vi "set Marker Control Mode.vi"(8 "error in (no error)":errorcluster, 9 "Marker Index":i32, 10 "Marker Mode":T1, 11 "FSV-40N in":refnum<class "FSV-40N.lvclass">) -> (0 "error out":errorcluster, 3 "FSV-40N out":refnum<class "FSV-40N.lvclass">)   [LabVIEW 2023, in "Spectrum Analyzer.lvlib" / "FSV-40N.lvclass"]
uses:
  FSV-40N.lvclass
  FSV-40N.lvclass/FSV-40N.ctl
  TYPE DEFINITION/TYPE Marker Control Mode.ctl
  Spectrum Analyzer.lvlib
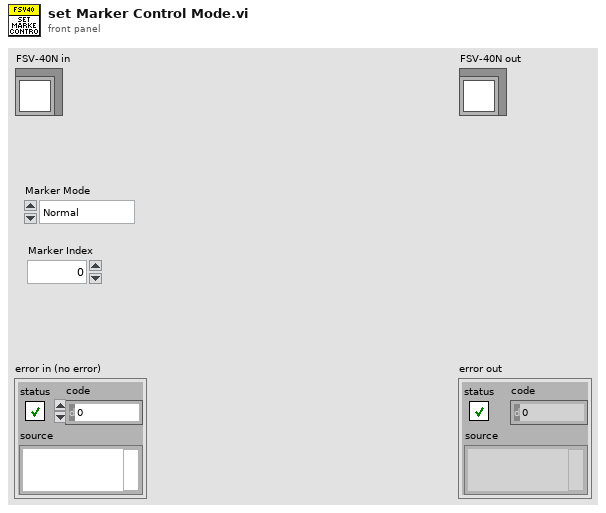
[diagram p1: front panel]
types:
  T1 = typedef "Spectrum Analyzer.lvlib/TYPE Marker Control Mode.ctl" = enum16{"Normal", "Delta", "Off"}
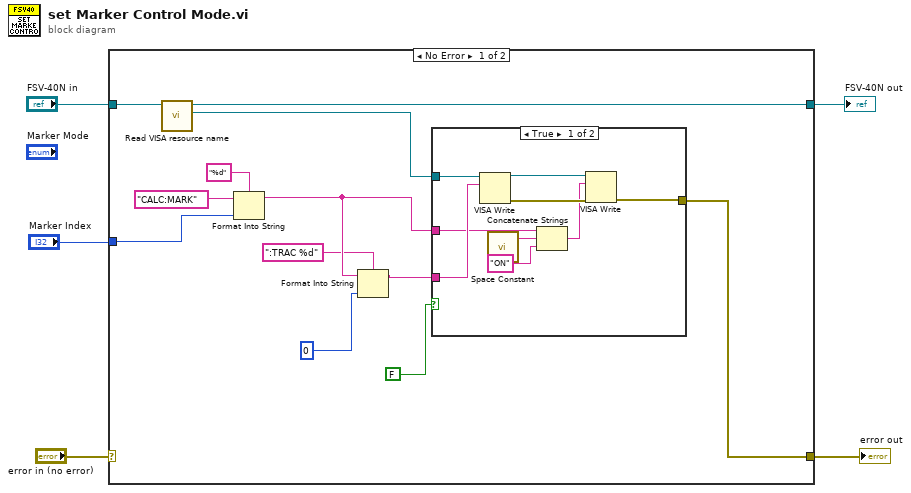
[diagram p0: block diagram]
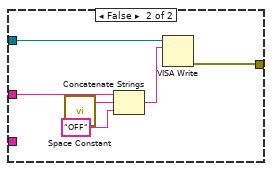
[diagram p2: hidden frame]
diagram:
  n1 = case shown="No Error" "error in (no error)" {
    selector: "error in (no error)" -> [_ w33]
    tunnel: "FSV-40N in" -> [w17 w34]
    tunnel: [w15 w34] -> w4
    tunnel: [w14 w33] -> w2
    tunnel: "Marker Index" -> [w11 _]
    frame No Error {
      n2 = call "Read VISA resource name.vi"("FSV-40N in"=w17) -> ("VISA resource name"=w16:refnum<visa-resource-name>, "FSV-40N out"=w15:refnum<class "FSV-40N.lvclass">)  [unwired: 8 in, 1 out]
      n3 = Format Into String(format string="%d", initial string="CALC:MARK" ("string"), w11) -> (resulting string=w10:string)  [unwired: 1 in, 1 out]
      n4 = Format Into String(format string=":TRAC %d" ("string"), initial string=w10, 0 ("input 1")) -> (resulting string=w9:string)  [unwired: 1 in, 1 out]
      n5 = case shown="True" FALSE {
        tunnel: w16 -> [w26 w32]
        tunnel: [w18 w27] -> w14
        tunnel: w9 -> [w23 _]
        tunnel: w10 -> [w22 w31]
        frame True {
          n6 = VISA Write(VISA resource name=w26, write buffer=w23) -> (VISA resource name out=w25:refnum<visa-resource-name>, error out=w24:errorcluster)  [unwired: 1 in, 1 out]
          n7 = call <vilib>:"Space Constant.vi"() -> ("String"=w21:string)
          n8 = Concatenate Strings(w22, w21, "ON" ("string")) -> (w19:string)
          n9 = VISA Write(VISA resource name=w25, write buffer=w19, error in (no error)=w24) -> (error out=w18:errorcluster)  [unwired: 2 out]
        }
        frame False {
          n10 = call <vilib>:"Space Constant.vi"() -> ("String"=w30:string)
          n11 = Concatenate Strings(w31, w30, "OFF" ("string")) -> (w28:string)
          n12 = VISA Write(VISA resource name=w32, write buffer=w28) -> (error out=w27:errorcluster)  [unwired: 1 in, 2 out]
        }
      }
    }
    frame Error {
    }
  }
  "error out" <- w2
  "FSV-40N out" <- w4
